vi "CSE - Close Instance.vi"(6 "error in":errorcluster, 9 "CSE RefNum":T1) -> (0 "error out":errorcluster, 1 "destroyed":bool, 3 "dup CSE RefNum":T1)   [LabVIEW 2021]
doc: "This VI closes the specified CSE instance context. If the context is dynamically created, the VI completely destroys it. If the context is static, the VI reinitializes it to reduce its memory footprint. Refer to the VI help for more details.\n\n<b>CSE RefNum</b> must contain a reference to a CSE instance context.\n\n::: CalcExpress Toolkit :::\nCopyright (c) 2000-2026 Konstantin Shifershteyn. All rights reserved."
uses:
  CSE Instance RefNum.ctl
  cersrc/celveng32.dll
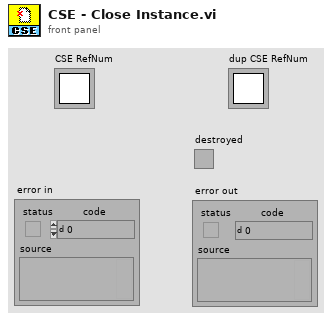
[diagram p1: front panel]
types:
  T1 = typedef "CSE Instance RefNum.ctl" = refnum<k1>
  T2 = enum16{"get RefNum", "close Clones", "close RefNum", "close all RefNums", "update RefNums"}
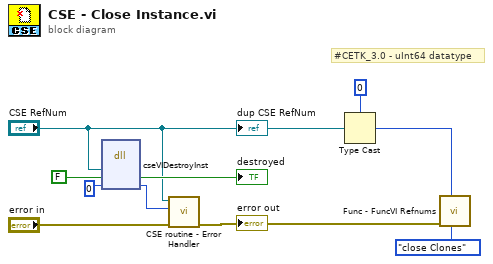
[diagram p0: block diagram]
diagram:
  # "#CETK_3.0 - uInt64 datatype"
  n1 = dll-call lib="C:/LV Projects/CalcExpress 40 LV2021/vi.lib/addons/CalcExpress/cersrc/celveng*.dll" fn="cseVIDestroyInst" ("viCESPDestroyInst")("iRef"="CSE RefNum", "destroyed"=FALSE, "erStat"=0) -> ("destroyed"=→"destroyed":bool, "erStat"=w7:i32)  [unwired: 5 in, 2 out]
  n2 = call "CSE routine - Error Handler.vi"("error in"="error in", "exec status"=w7, "CSE RefNum"="CSE RefNum") -> ("error out"=w2:errorcluster)  [unwired: 4 in, 2 out]
  "error out" <- w2
  n3 = Type Cast(type=u64 0, x="CSE RefNum") -> (*(type *) &x=w3:u64)
  n4 = call "Func - FuncVI Refnums.vi"("cmd (get)"=T2."close Clones", "Instance ID"=w3, "error in"=w2) -> ()  [unwired: 4 in, 5 out]
  "dup CSE RefNum" <- "CSE RefNum"
